vi "Joystick Configuration.vi"() -> ()   [LabVIEW 2021]
uses:
  <vilib>/Utility/inputDevices.llb/joystickAcquire.vi
  <vilib>/Utility/inputDevices.llb/closeJoystick.vi
panel:
  out "Joystick Status":bool
  in  "stop":bool
  out "axis info":T1
  out "button info":T2
  out "direction info":T3
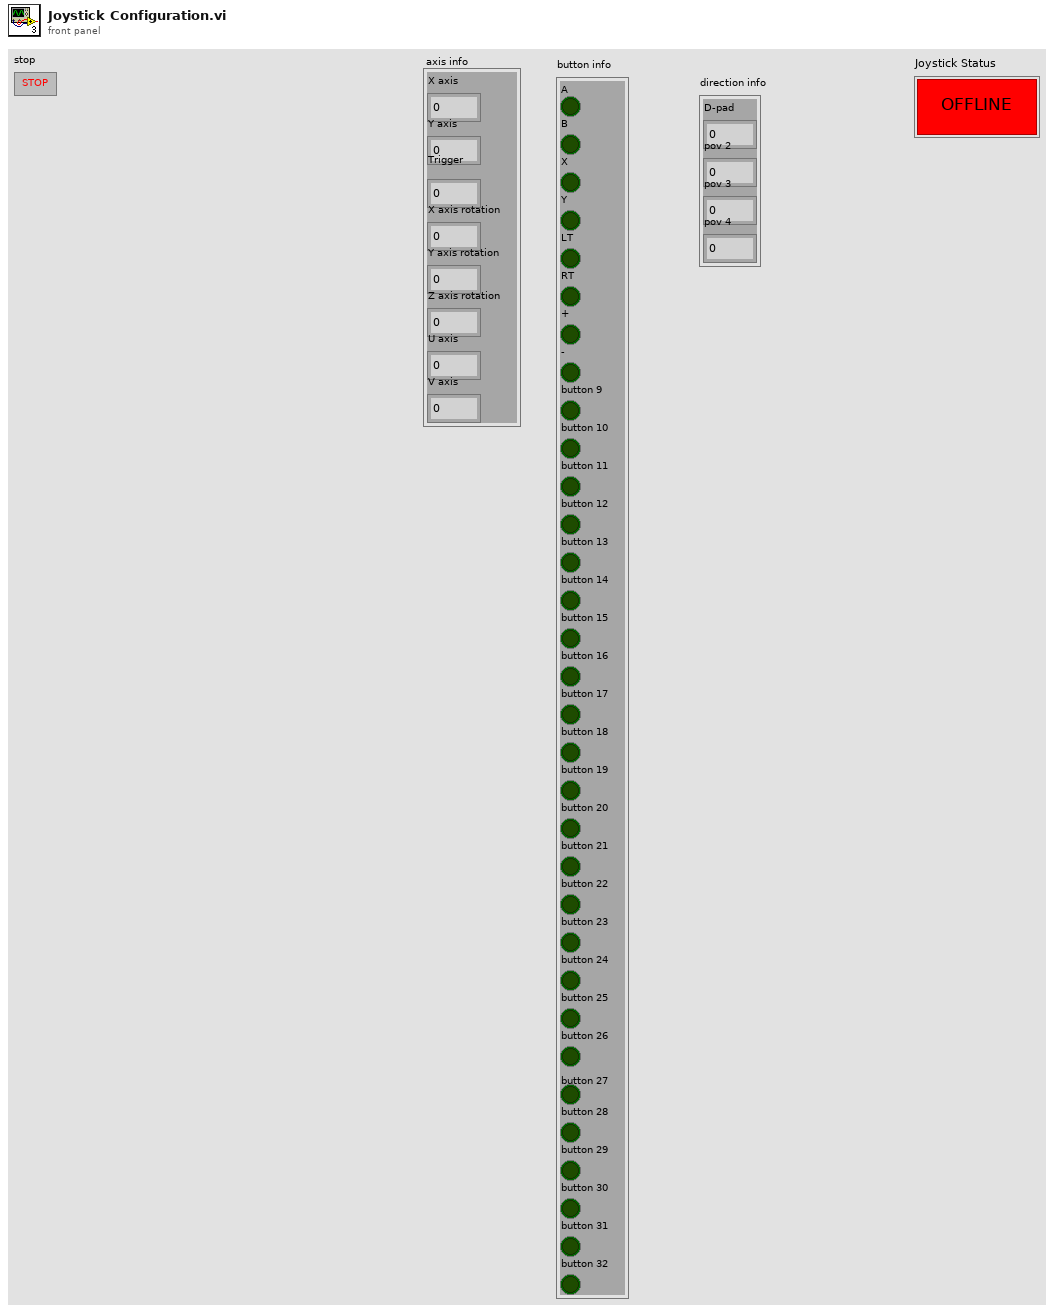
[diagram p1: front panel]
types:
  T1 = cluster{"X axis":i32, "Y axis":i32, "\nTrigger":i32, "X axis rotation":i32, "Y axis rotation":i32, "Z axis rotation":i32, "U axis":i32, "V axis":i32}
  T2 = cluster{"A":bool, "B":bool, "X":bool, "Y":bool, "LT":bool, "RT":bool, "+":bool, "-":bool, "button 9":bool, "button 10":bool, "button 11":bool, "button 12":bool, "button 13":bool, "button 14":bool, "button 15":bool, "button 16":bool, "button 17":bool, "button 18":bool, "button 19":bool, "button 20":bool, "button 21":bool, "button 22":bool, "button 23":bool, "button 24":bool, "button 25":bool, "button 26":bool, "button 27":bool, "button 28":bool, "button 29":bool, "button 30":bool, "button 31":bool, "button 32":bool}
  T3 = cluster{"D-pad":i32, "pov 2":i32, "pov 3":i32, "pov 4":i32}
  T4 = cluster{"X axis":i32, "Y axis":i32, "Z axis":i32, "X axis rotation":i32, "Y axis rotation":i32, "Z axis rotation":i32, "U axis":i32, "V axis":i32}
  T5 = cluster{"button 1":bool, "button 2":bool, "button 3":bool, "button 4":bool, "button 5":bool, "button 6":bool, "button 7":bool, "button 8":bool, "button 9":bool, "button 10":bool, "button 11":bool, "button 12":bool, "button 13":bool, "button 14":bool, "button 15":bool, "button 16":bool, "button 17":bool, "button 18":bool, "button 19":bool, "button 20":bool, "button 21":bool, "button 22":bool, "button 23":bool, "button 24":bool, "button 25":bool, "button 26":bool, "button 27":bool, "button 28":bool, "button 29":bool, "button 30":bool, "button 31":bool, "button 32":bool}
  T6 = cluster{"pov 1":i32, "pov 2":i32, "pov 3":i32, "pov 4":i32}
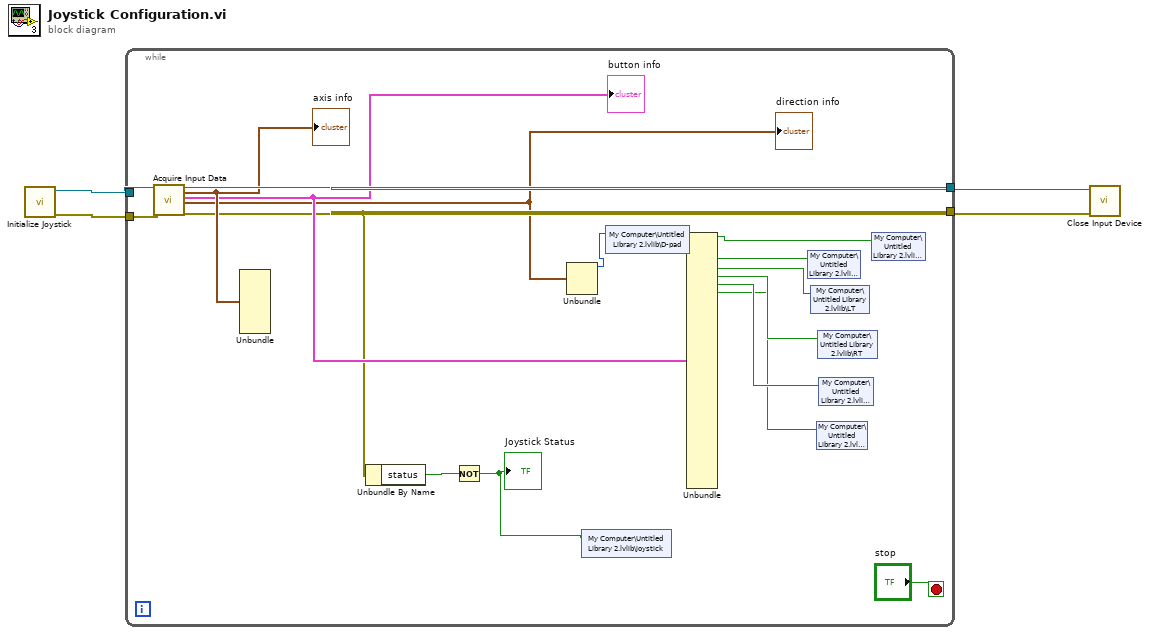
[diagram p0: block diagram]
diagram:
  n1 = call <vilib>:"Initialize Joystick.vi"() -> ("error out"=w3:errorcluster, "device ID"=w4:refnum<k1>)  [unwired: 10 in]
  n2 = while {
    tunnel: w4 -> [w21]
    tunnel: w3 -> [w20]
    tunnel: [w19] -> w2
    tunnel: [w14] -> w1
    stop <- "stop" stop-if-true
    n3 = call-poly <vilib>:"Acquire Input Data.vi"("device ID"=w21, "error in (no error)"=w20) -> ("device ID"=w19:refnum<k1>, "axis info"=w17:T4, "button info"=w16:T5, "direction info"=w15:T6, "error out"=w14:errorcluster)  [unwired: 13 in]
    "axis info" <- w17
    "button info" <- w16
    "direction info" <- w15
    n4 = Unbundle(w17) -> ()  [unwired: 8 out]
    n5 = Unbundle By Name(w14) -> ("status"=w13:bool)
    n6 = Not(x=w13) -> (.not. x?=w12:bool)
    "Joystick Status" <- w12
    n7 = Unbundle(w15) -> ("pov 1"=w11:i32)  [unwired: 3 out]
    n8 = shared-variable "My Computer\\Untitled Library 2.lvlib\\joystick"(w12) -> ()  [unwired: 1 in, 1 out]
    n9 = shared-variable "My Computer\\Untitled Library 2.lvlib\\D-pad"(w11) -> ()  [unwired: 1 in, 1 out]
    n10 = Unbundle(w16) -> ("button 1"=w7:bool, "button 4"=w10:bool, "button 5"=w9:bool, "button 6"=w8:bool, "button 7"=w6:bool, "button 8"=w5:bool)  [unwired: 26 out]
    n11 = shared-variable "My Computer\\Untitled Library 2.lvlib\\Y"(w10) -> ()  [unwired: 1 in, 1 out]
    n12 = shared-variable "My Computer\\Untitled Library 2.lvlib\\LT"(w9) -> ()  [unwired: 1 in, 1 out]
    n13 = shared-variable "My Computer\\Untitled Library 2.lvlib\\-"(w5) -> ()  [unwired: 1 in, 1 out]
    n14 = shared-variable "My Computer\\Untitled Library 2.lvlib\\RT"(w8) -> ()  [unwired: 1 in, 1 out]
    n15 = shared-variable "My Computer\\Untitled Library 2.lvlib\\+"(w6) -> ()  [unwired: 1 in, 1 out]
    n16 = shared-variable "My Computer\\Untitled Library 2.lvlib\\A"(w7) -> ()  [unwired: 1 in, 1 out]
  }
  n17 = call-poly <vilib>:"Close Input Device.vi"("error in (no error)"=w1, "device ID"=w2) -> ()  [unwired: 8 in, 1 out]
